vi "Check.vi"(7 "VolatusAPI":refnum<class "VolatusAPI.lvclass">, 8 "error in (no error)":errorcluster, 11 "cRIO Power Status EStop in":refnum<class "cRIO Power Status EStop.lvclass">) -> (0 "error out":errorcluster, 2 "Active":bool, 3 "cRIO Power Status EStop out":refnum<class "cRIO Power Status EStop.lvclass">)   [LabVIEW 2025, in "VolatusControl.lvlib" / "cRIO Power Status EStop.lvclass"]
uses:
  cRIO Power Status EStop.lvclass
  Volatus/VolatusAPI/VolatusAPI.lvclass
  cRIO Power Status EStop.lvclass/cRIO Power Status EStop.ctl
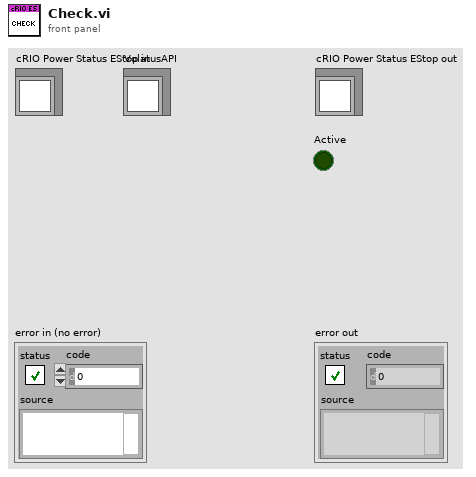
[diagram p1: front panel]
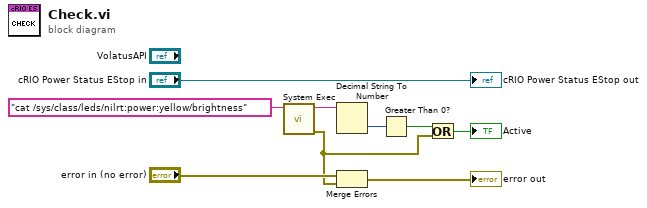
[diagram p0: block diagram]
diagram:
  n1 = call <vilib>:"System Exec.vi"("command line"="cat /sys/class/leds/nilrt:power:yellow/brightness") -> ("error out"=w1:errorcluster, "standard output"=w3:string)  [unwired: 7 in, 2 out]
  n2 = Decimal String To Number(string=w3) -> (number=w7:i32)  [unwired: 2 in, 1 out]
  n3 = Merge Errors("error in (no error)", w1) -> (→"error out":errorcluster)
  n4 = Greater Than 0?(x=w7) -> (x > 0?=w6:bool)
  n5 = Or(x=w6, y=w1) -> (x .or. y?=→"Active":bool)
  "cRIO Power Status EStop out" <- "cRIO Power Status EStop in"
